vi "Run VIA.vi"(4 "MaxBuildVer":string, 6 "Buildlog":path, 7 "Build number":u32, 8 "error in (no error)":errorcluster, 10 "args":string[](array[string]), 11 "VI Path":path) -> (0 "error out":errorcluster)   [LabVIEW 2010]
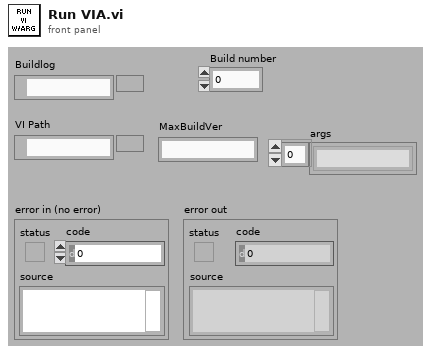
[diagram p1: front panel]
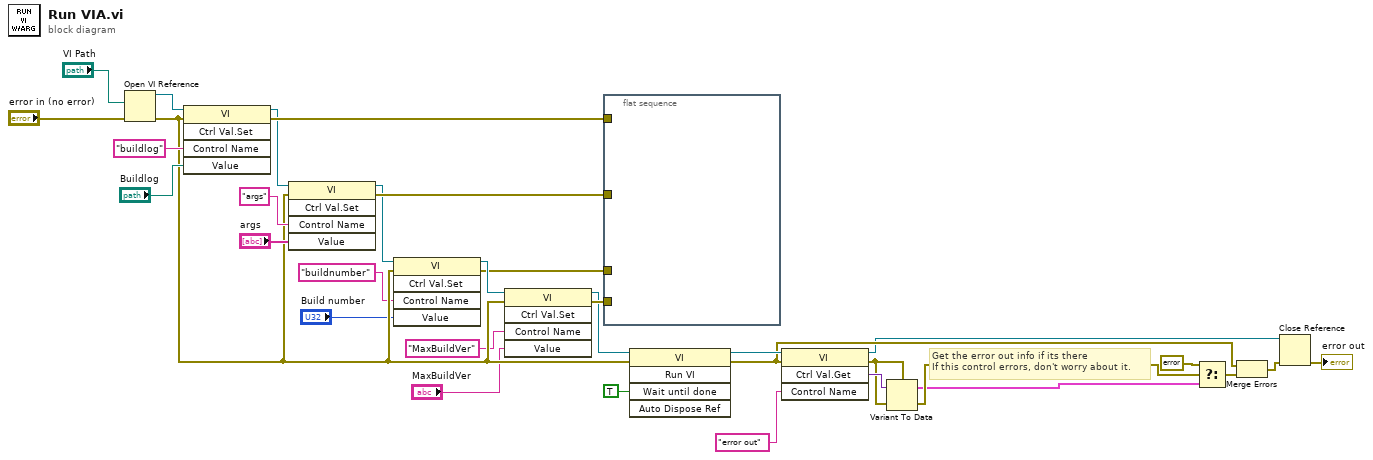
[diagram p0: block diagram]
diagram:
  # "Get the error out info if its there\nIf this control errors, don't worry about it."
  n1 = Open VI Reference(vi path="VI Path", error in (no error)="error in (no error)") -> (vi reference=w17:refnum<vi>, error out=w6:errorcluster)  [unwired: 4 in]
  n2 = invoke class="VI" method="Ctrl Val.Set"(reference=w17, error in=w6, "Control Name"="buildlog", "Value"="Buildlog") -> (reference out=w14:refnum<vi>, error out=w15:errorcluster)  [unwired: 1 in, 3 out]
  n3 = invoke class="VI" method="Ctrl Val.Set"(reference=w14, error in=w6, "Control Name"="args", "Value"="args") -> (reference out=w7:refnum<vi>, error out=w13:errorcluster)  [unwired: 1 in, 3 out]
  n4 = invoke class="VI" method="Ctrl Val.Set"(reference=w7, error in=w6, "Control Name"="buildnumber", "Value"="Build number") -> (reference out=w10:refnum<vi>, error out=w9:errorcluster)  [unwired: 1 in, 3 out]
  n5 = invoke class="VI" method="Ctrl Val.Set"(reference=w10, error in=w6, "Control Name"="MaxBuildVer", "Value"="MaxBuildVer") -> (reference out=w1:refnum<vi>, error out=w8:errorcluster)  [unwired: 1 in, 3 out]
  n6 = flat-sequence {
    tunnel: w15 -> [_]
    tunnel: w13 -> [_]
    tunnel: w9 -> [_]
    tunnel: w8 -> [_]
    frame #0 {
    }
  }
  n7 = invoke class="VI" method="Run VI"(reference=w1, error in=w6, "Wait until done"=TRUE ("Wait Until Done")) -> (reference out=w30:refnum<vi>, error out=w23:errorcluster)  [unwired: 2 in, 3 out]
  n8 = invoke class="VI" method="Ctrl Val.Get"(reference=w30, error in=w23, "Control Name"="error out") -> (reference out=w19:refnum<vi>, error out=w27:errorcluster, "Get Control Value Variant"=w28:variant)  [unwired: 1 in, 1 out]
  n9 = Variant To Data(error in=w27, Variant=w28, type=w27) -> (error out=w26:errorcluster, data=w24:cluster{})
  n10 = Select(t=errorcluster {"status"=FALSE, "code"=0, "source"=""}, s=w26, f=w24) -> (s? t:f=w22:errorcluster)
  n11 = Merge Errors(w23, w22) -> (w21:errorcluster)
  n12 = Close Reference(reference=w19, error in (no error)=w21) -> (error out=→"error out":errorcluster)
